vi "init CE SEM Full Mask Table.vi"(8 "error in (no error)":errorcluster, 11 "SA Measurement in":refnum<class "SA Measurement.lvclass">) -> (0 "error out":errorcluster, 3 "SA Measurement out":refnum<class "SA Measurement.lvclass">)   [LabVIEW 2023, in "Spectrum Analyzer.lvlib" / "SA Measurement.lvclass"]
uses:
  SA Measurement.lvclass
  SA Measurement.lvclass/SA Measurement.ctl
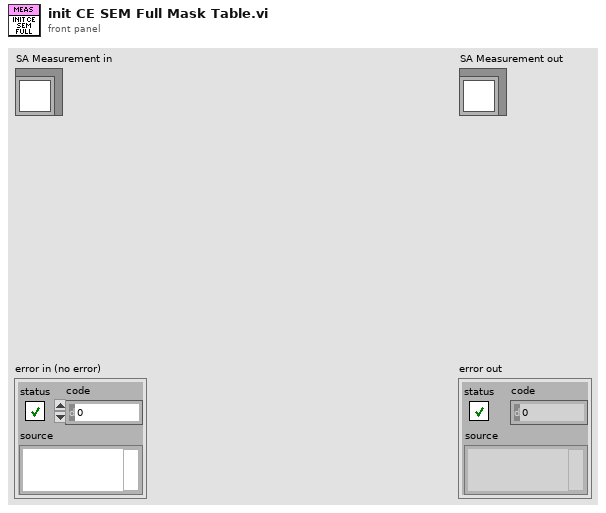
[diagram p1: front panel]
types:
  T1 = cluster{"Mask Case":enum16{"Full", "Case 1", "Case 2", "Case 3", "Case 1+2"}, "BW_N":dbl, "BW_M":dbl}[]
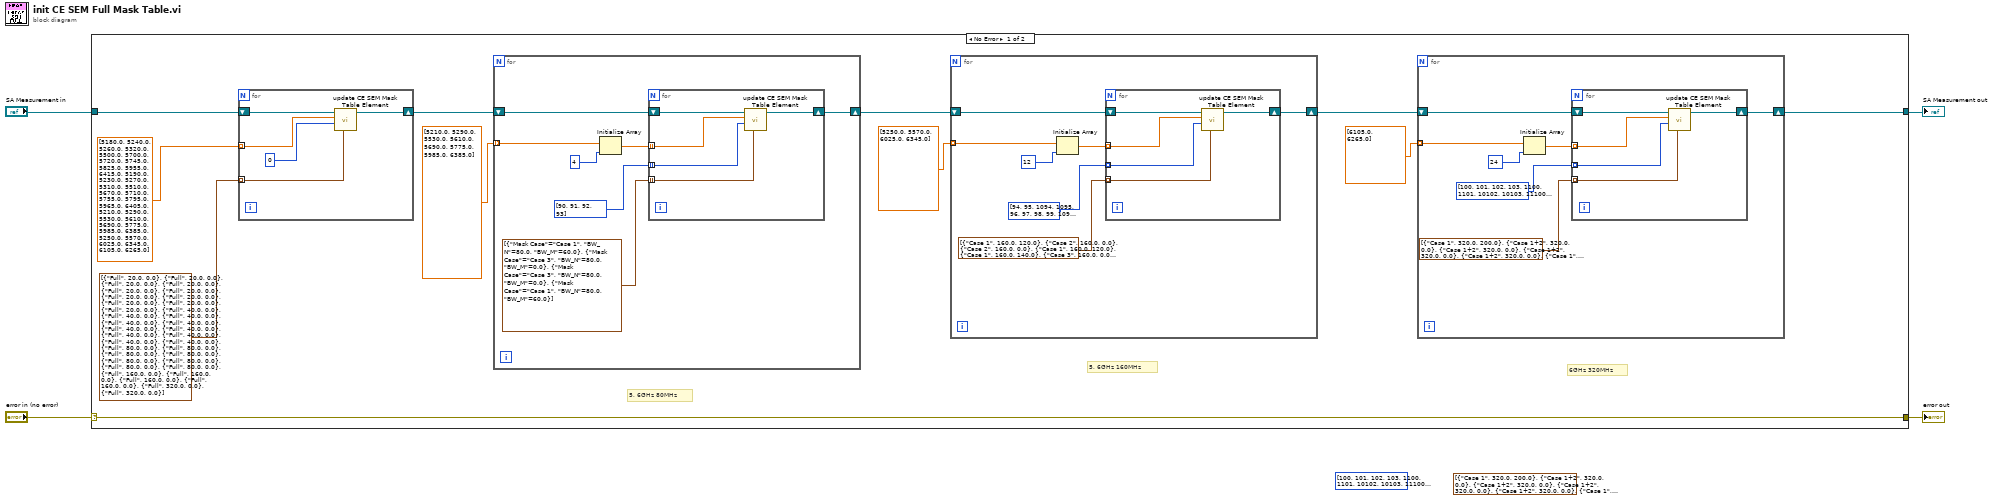
[diagram p0: block diagram]
diagram:
  (unwired) T1 [{"Mask Case"=enum."Case 1", "BW_N"=320.0, "BW_M"=200.0}, {"Mask Case"=enum."Case 1+2", "BW_N"=320.0, "BW_M"=0.0}, {"Mask Case"=enum."Case 1+2", "BW_N"=320.0, "BW_M"=0.0}, {"Mask Case"=enum."Case 1+2", "BW_N"=320.0, "BW_M"=0.0}, {"Mask Case"=enum."Case 1+2", "BW_N"=320.0, "BW_M"=0.0}, {"Mask Case"=enum."Case 1", "BW_N"=320.0, "BW_M"=200.0}, {"Mask Case"=enum."Case 1", "BW_N"=320.0, "BW_M"=200.0}, {"Mask Case"=enum."Case 1+2", "BW_N"=320.0, "BW_M"=0.0}, {"Mask Case"=enum."Case 1+2", "BW_N"=320.0, "BW_M"=0.0}, {"Mask Case"=enum."Case 1+2", "BW_N"=320.0, "BW_M"=0.0}, {"Mask Case"=enum."Case 1+2", "BW_N"=320.0, "BW_M"=0.0}, {"Mask Case"=enum."Case 1", "BW_N"=320.0, "BW_M"=200.0}, {"Mask Case"=enum."Case 1", "BW_N"=320.0, "BW_M"=240.0}, {"Mask Case"=enum."Case 2", "BW_N"=320.0, "BW_M"=0.0}, {"Mask Case"=enum."Case 2", "BW_N"=320.0, "BW_M"=0.0}, {"Mask Case"=enum."Case 1", "BW_N"=320.0, "BW_M"=240.0}, {"Mask Case"=enum."Case 1", "BW_N"=320.0, "BW_M"=280.0}, {"Mask Case"=enum."Case 2", "BW_N"=320.0, "BW_M"=0.0}, {"Mask Case"=enum."Case 2", "BW_N"=320.0, "BW_M"=0.0}, {"Mask Case"=enum."Case 2", "BW_N"=320.0, "BW_M"=0.0}, {"Mask Case"=enum."Case 2", "BW_N"=320.0, "BW_M"=0.0}, {"Mask Case"=enum."Case 2", "BW_N"=320.0, "BW_M"=0.0}, {"Mask Case"=enum."Case 2", "BW_N"=320.0, "BW_M"=0.0}, {"Mask Case"=enum."Case 1", "BW_N"=320.0, "BW_M"=280.0}] ("Mask Type Info")
  (unwired) i32[] [100, 101, 102, 103, 1100, 1101, 10102, 10103, 11100, 11101, 11102, 11103, 104, 1104, 10104, 11104, 105, 106, 1105, 1106, 10105, 10106, 11105, 11106] ("RU Type (0=Full Mask)")
  n1 = case shown="No Error" "error in (no error)" {
    selector: "error in (no error)" -> [w15 w58]
    tunnel: [w15 w58] -> w3
    tunnel: [w5 w57] -> w1
    tunnel: "SA Measurement in" -> [w14 w57]
    frame No Error {
      # "6GHz 320MHz"
      # "5, 6GHz 80MHz"
      # "5, 6GHz 160MHz"
      n2 = for {
        tunnel: dbl[] [5180.0, 5240.0, 5260.0, 5320.0, 5500.0, 5700.0, 5720.0, 5745.0, 5825.0, 5955.0, 6415.0, 5190.0, 5230.0, 5270.0, 5310.0, 5510.0, 5670.0, 5710.0, 5755.0, 5795.0, 5965.0, 6405.0, 5210.0, 5290.0, 5530.0, 5610.0, 5690.0, 5775.0, 5985.0, 6385.0, 5250.0, 5570.0, 6025.0, 6345.0, 6105.0, 6265.0] ("key") -> [w54] mode=indexing
        tunnel: T1 [{"Mask Case"=enum."Full", "BW_N"=20.0, "BW_M"=0.0}, {"Mask Case"=enum."Full", "BW_N"=20.0, "BW_M"=0.0}, {"Mask Case"=enum."Full", "BW_N"=20.0, "BW_M"=0.0}, {"Mask Case"=enum."Full", "BW_N"=20.0, "BW_M"=0.0}, {"Mask Case"=enum."Full", "BW_N"=20.0, "BW_M"=0.0}, {"Mask Case"=enum."Full", "BW_N"=20.0, "BW_M"=0.0}, {"Mask Case"=enum."Full", "BW_N"=20.0, "BW_M"=0.0}, {"Mask Case"=enum."Full", "BW_N"=20.0, "BW_M"=0.0}, {"Mask Case"=enum."Full", "BW_N"=20.0, "BW_M"=0.0}, {"Mask Case"=enum."Full", "BW_N"=20.0, "BW_M"=0.0}, {"Mask Case"=enum."Full", "BW_N"=20.0, "BW_M"=0.0}, {"Mask Case"=enum."Full", "BW_N"=40.0, "BW_M"=0.0}, {"Mask Case"=enum."Full", "BW_N"=40.0, "BW_M"=0.0}, {"Mask Case"=enum."Full", "BW_N"=40.0, "BW_M"=0.0}, {"Mask Case"=enum."Full", "BW_N"=40.0, "BW_M"=0.0}, {"Mask Case"=enum."Full", "BW_N"=40.0, "BW_M"=0.0}, {"Mask Case"=enum."Full", "BW_N"=40.0, "BW_M"=0.0}, {"Mask Case"=enum."Full", "BW_N"=40.0, "BW_M"=0.0}, {"Mask Case"=enum."Full", "BW_N"=40.0, "BW_M"=0.0}, {"Mask Case"=enum."Full", "BW_N"=40.0, "BW_M"=0.0}, {"Mask Case"=enum."Full", "BW_N"=40.0, "BW_M"=0.0}, {"Mask Case"=enum."Full", "BW_N"=40.0, "BW_M"=0.0}, {"Mask Case"=enum."Full", "BW_N"=80.0, "BW_M"=0.0}, {"Mask Case"=enum."Full", "BW_N"=80.0, "BW_M"=0.0}, {"Mask Case"=enum."Full", "BW_N"=80.0, "BW_M"=0.0}, {"Mask Case"=enum."Full", "BW_N"=80.0, "BW_M"=0.0}, {"Mask Case"=enum."Full", "BW_N"=80.0, "BW_M"=0.0}, {"Mask Case"=enum."Full", "BW_N"=80.0, "BW_M"=0.0}, {"Mask Case"=enum."Full", "BW_N"=80.0, "BW_M"=0.0}, {"Mask Case"=enum."Full", "BW_N"=80.0, "BW_M"=0.0}, {"Mask Case"=enum."Full", "BW_N"=160.0, "BW_M"=0.0}, {"Mask Case"=enum."Full", "BW_N"=160.0, "BW_M"=0.0}, {"Mask Case"=enum."Full", "BW_N"=160.0, "BW_M"=0.0}, {"Mask Case"=enum."Full", "BW_N"=160.0, "BW_M"=0.0}, {"Mask Case"=enum."Full", "BW_N"=320.0, "BW_M"=0.0}, {"Mask Case"=enum."Full", "BW_N"=320.0, "BW_M"=0.0}] ("Mask Type Info") -> [w53] mode=indexing
        shift-right: [w52] -> w11
        shift-left: w14 -> [w56]
        n3 = call "update CE SEM Mask Table Element.vi"("Mask Type Info"=w53, "RU Type (0=Full Mask)"=0, "Center Freq"=w54, "SA Measurement in"=w56) -> ("SA Measurement out"=w52:refnum<class "SA Measurement.lvclass">)  [unwired: 6 in, 1 out]
      }
      n4 = for {
        tunnel: dbl[] [5210.0, 5290.0, 5530.0, 5610.0, 5690.0, 5775.0, 5985.0, 6385.0] ("element") -> [w43] mode=indexing
        shift-right: [w45] -> w8
        shift-left: w11 -> [w46]
        n5 = Initialize Array(w43, 4 ("dimension size")) -> (w41:dbl[])
        n6 = for {
          tunnel: w41 -> [w50] mode=indexing
          tunnel: T1 [{"Mask Case"=enum."Case 1", "BW_N"=80.0, "BW_M"=60.0}, {"Mask Case"=enum."Case 3", "BW_N"=80.0, "BW_M"=0.0}, {"Mask Case"=enum."Case 3", "BW_N"=80.0, "BW_M"=0.0}, {"Mask Case"=enum."Case 1", "BW_N"=80.0, "BW_M"=60.0}] ("Mask Type Info") -> [w49] mode=indexing
          shift-right: [w48] -> w45
          shift-left: w46 -> [w51]
          tunnel: i32[] [90, 91, 92, 93] ("RU Type (0=Full Mask)") -> [w47] mode=indexing
          n7 = call "update CE SEM Mask Table Element.vi"("Mask Type Info"=w49, "RU Type (0=Full Mask)"=w47, "Center Freq"=w50, "SA Measurement in"=w51) -> ("SA Measurement out"=w48:refnum<class "SA Measurement.lvclass">)  [unwired: 6 in, 1 out]
        }
      }
      n8 = for {
        tunnel: dbl[] [5250.0, 5570.0, 6025.0, 6345.0] ("element") -> [w32] mode=indexing
        shift-right: [w33] -> w6
        shift-left: w8 -> [w34]
        n9 = Initialize Array(w32, 12 ("dimension size")) -> (w30:dbl[])
        n10 = for {
          tunnel: w30 -> [w38] mode=indexing
          tunnel: T1 [{"Mask Case"=enum."Case 1", "BW_N"=160.0, "BW_M"=120.0}, {"Mask Case"=enum."Case 2", "BW_N"=160.0, "BW_M"=0.0}, {"Mask Case"=enum."Case 2", "BW_N"=160.0, "BW_M"=0.0}, {"Mask Case"=enum."Case 1", "BW_N"=160.0, "BW_M"=120.0}, {"Mask Case"=enum."Case 1", "BW_N"=160.0, "BW_M"=140.0}, {"Mask Case"=enum."Case 3", "BW_N"=160.0, "BW_M"=0.0}, {"Mask Case"=enum."Case 3", "BW_N"=160.0, "BW_M"=0.0}, {"Mask Case"=enum."Case 3", "BW_N"=160.0, "BW_M"=0.0}, {"Mask Case"=enum."Case 3", "BW_N"=160.0, "BW_M"=0.0}, {"Mask Case"=enum."Case 3", "BW_N"=160.0, "BW_M"=0.0}, {"Mask Case"=enum."Case 3", "BW_N"=160.0, "BW_M"=0.0}, {"Mask Case"=enum."Case 1", "BW_N"=160.0, "BW_M"=140.0}] ("Mask Type Info") -> [w37] mode=indexing
          shift-right: [w36] -> w33
          shift-left: w34 -> [w39]
          tunnel: i32[] [94, 95, 1094, 1095, 96, 97, 98, 99, 1096, 1097, 1098, 1099] ("RU Type (0=Full Mask)") -> [w35] mode=indexing
          n11 = call "update CE SEM Mask Table Element.vi"("Mask Type Info"=w37, "RU Type (0=Full Mask)"=w35, "Center Freq"=w38, "SA Measurement in"=w39) -> ("SA Measurement out"=w36:refnum<class "SA Measurement.lvclass">)  [unwired: 6 in, 1 out]
        }
      }
      n12 = for {
        tunnel: dbl[] [6105.0, 6265.0] ("element") -> [w20] mode=indexing
        shift-right: [w21] -> w5
        shift-left: w6 -> [w22]
        n13 = Initialize Array(w20, 24 ("dimension size")) -> (w18:dbl[])
        n14 = for {
          tunnel: w18 -> [w26] mode=indexing
          tunnel: T1 [{"Mask Case"=enum."Case 1", "BW_N"=320.0, "BW_M"=200.0}, {"Mask Case"=enum."Case 1+2", "BW_N"=320.0, "BW_M"=0.0}, {"Mask Case"=enum."Case 1+2", "BW_N"=320.0, "BW_M"=0.0}, {"Mask Case"=enum."Case 1+2", "BW_N"=320.0, "BW_M"=0.0}, {"Mask Case"=enum."Case 1+2", "BW_N"=320.0, "BW_M"=0.0}, {"Mask Case"=enum."Case 1", "BW_N"=320.0, "BW_M"=200.0}, {"Mask Case"=enum."Case 1", "BW_N"=320.0, "BW_M"=200.0}, {"Mask Case"=enum."Case 1+2", "BW_N"=320.0, "BW_M"=0.0}, {"Mask Case"=enum."Case 1+2", "BW_N"=320.0, "BW_M"=0.0}, {"Mask Case"=enum."Case 1+2", "BW_N"=320.0, "BW_M"=0.0}, {"Mask Case"=enum."Case 1+2", "BW_N"=320.0, "BW_M"=0.0}, {"Mask Case"=enum."Case 1", "BW_N"=320.0, "BW_M"=200.0}, {"Mask Case"=enum."Case 1", "BW_N"=320.0, "BW_M"=240.0}, {"Mask Case"=enum."Case 2", "BW_N"=320.0, "BW_M"=0.0}, {"Mask Case"=enum."Case 2", "BW_N"=320.0, "BW_M"=0.0}, {"Mask Case"=enum."Case 1", "BW_N"=320.0, "BW_M"=240.0}, {"Mask Case"=enum."Case 1", "BW_N"=320.0, "BW_M"=280.0}, {"Mask Case"=enum."Case 2", "BW_N"=320.0, "BW_M"=0.0}, {"Mask Case"=enum."Case 2", "BW_N"=320.0, "BW_M"=0.0}, {"Mask Case"=enum."Case 2", "BW_N"=320.0, "BW_M"=0.0}, {"Mask Case"=enum."Case 2", "BW_N"=320.0, "BW_M"=0.0}, {"Mask Case"=enum."Case 2", "BW_N"=320.0, "BW_M"=0.0}, {"Mask Case"=enum."Case 2", "BW_N"=320.0, "BW_M"=0.0}, {"Mask Case"=enum."Case 1", "BW_N"=320.0, "BW_M"=280.0}] ("Mask Type Info") -> [w25] mode=indexing
          shift-right: [w24] -> w21
          shift-left: w22 -> [w27]
          tunnel: i32[] [100, 101, 102, 103, 1100, 1101, 10102, 10103, 11100, 11101, 11102, 11103, 104, 1104, 10104, 11104, 105, 106, 1105, 1106, 10105, 10106, 11105, 11106] ("RU Type (0=Full Mask)") -> [w23] mode=indexing
          n15 = call "update CE SEM Mask Table Element.vi"("Mask Type Info"=w25, "RU Type (0=Full Mask)"=w23, "Center Freq"=w26, "SA Measurement in"=w27) -> ("SA Measurement out"=w24:refnum<class "SA Measurement.lvclass">)  [unwired: 6 in, 1 out]
        }
      }
    }
    frame Error {
    }
  }
  "error out" <- w3
  "SA Measurement out" <- w1
